vi "Tree Rows from Delimited String Array_csm.vi"(8 "Use Child Only? (F)":bool, 9 "Default Symbol":i32, 10 "Delimiter":string="\\", 11 "Items (Delimited)":string[][](array[string])) -> (2 "Parent Tag Added[]":string[](array[string]), 3 "Item to Add[]":T1(array[cluster]))   [LabVIEW 2017, in "csm-ui-support.lvlib"]
uses:
  csm-ui-support.lvlib
panel:
  out "Index":i32
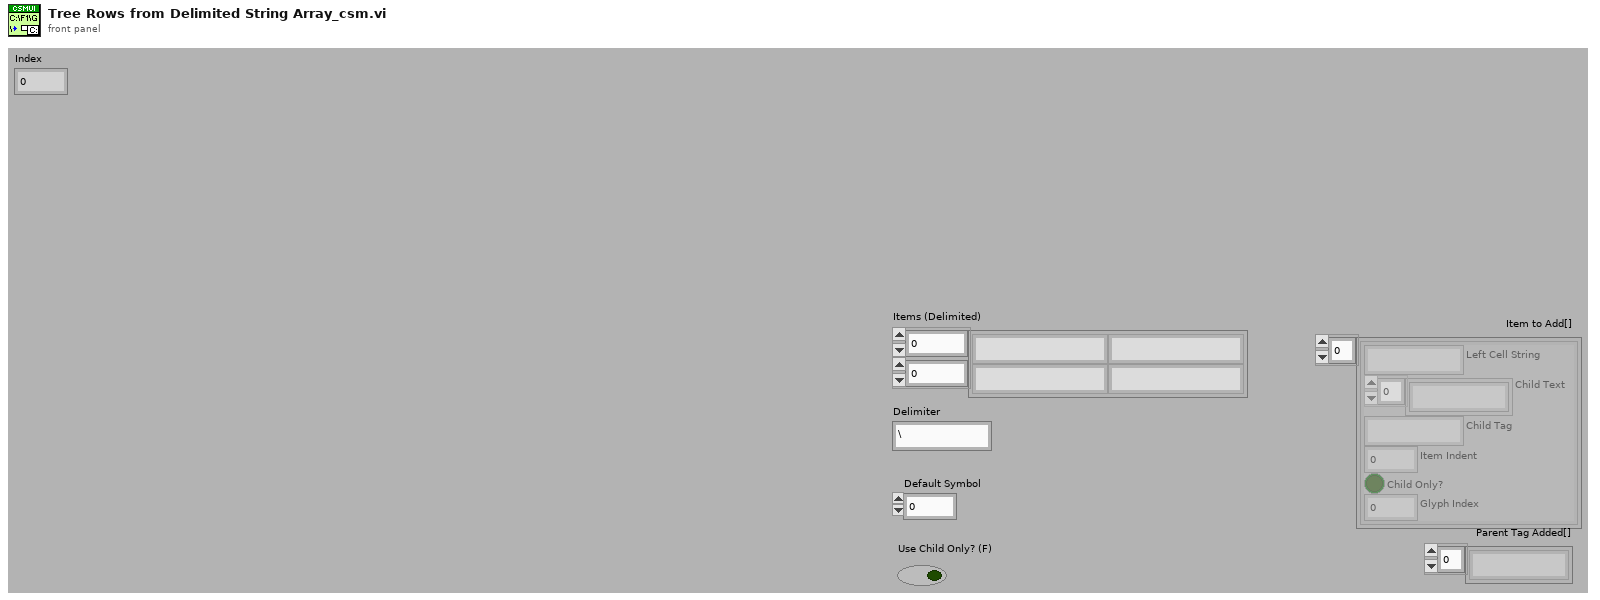
[diagram p1: front panel]
types:
  T1 = cluster{"Left Cell String":string, "Child Text":string[], "Child Tag":string, "Item Indent":i32, "Child Only?":bool, "Glyph Index":i32}[]
  T2 = cluster{"Left Cell String":string, "Child Text":string[], "Child Tag":string, "Item Indent":i32, "Child Only?":bool, "Glyph Index":i32}
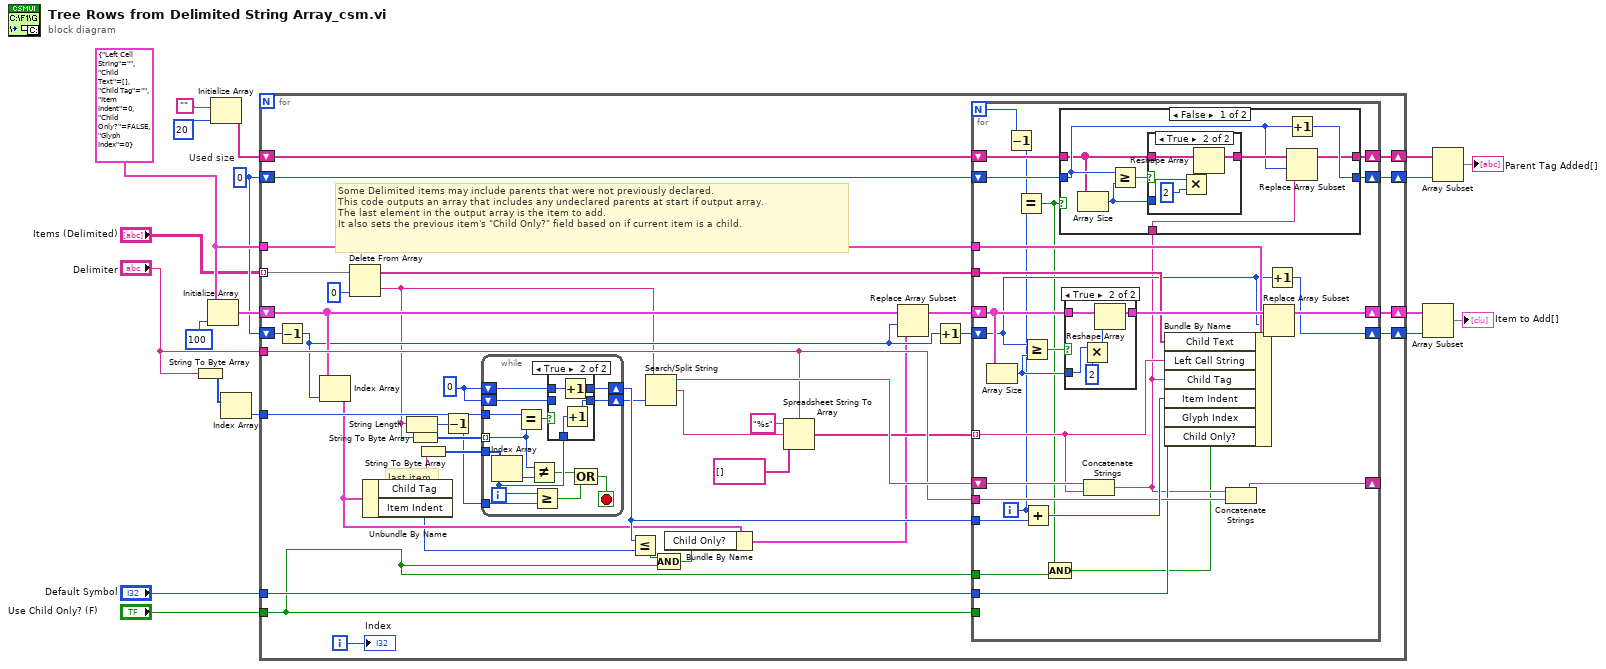
[diagram p0: block diagram]
diagram:
  w2 = 0  # Used size
  w8 = T2 {"Left Cell String"="", "Child Text"=[], "Child Tag"="", "Item Indent"=0, "Child Only?"=FALSE, "Glyph Index"=0} ("Item")
  n1 = String To Byte Array(string="Delimiter") -> (unsigned byte array=w18:u8[])
  n2 = Initialize Array(w8, 100 ("dimension size")) -> (w15:T1)
  n3 = Initialize Array("", 20 ("dimension size")) -> (w14:string[])
  n4 = Index Array(array=w18) -> (element=w19:u8)  [unwired: 1 in]
  n5 = for {
    shift-right: [w56] -> w17
    shift-left: w2 -> [w45]
    shift-right: [w57] -> w16
    shift-left: w15 -> [w46]
    tunnel: "Items (Delimited)" -> [w58] mode=indexing
    tunnel: "Delimiter" -> [w50]
    tunnel: w8 -> [w54]
    tunnel: w19 -> [w52]
    tunnel: "Default Symbol" -> [w47]
    tunnel: "Use Child Only? (F)" -> [w41]
    shift-right: [w38] -> w11
    shift-left: w14 -> [w40]
    shift-right: [w37] -> w10
    shift-left: w2 -> [w39]
    i -> [w53]
    w31 = 0
    # "last item"
    # "Some Delimited items may include parents that were not previously declared.\nThis code outputs an array that includes any undeclared parents at start if output array.\nThe last element in the output array is the item to add.\nIt also sets the previous item's \"Child Only?\" field based on if current item is a child."
    n6 = Decrement(x=w45) -> (x-1=w44:i32)
    n7 = Index Array(array=w46, index=w44) -> (element=w29:T2)
    n8 = Delete From Array(array=w58, index=0) -> (deleted portion=w24:string, array with subset deleted=w55:string[])  [unwired: 1 in]
    n9 = Unbundle By Name(w29) -> ("Child Tag"=w35:string, "Item Indent"=w26:i32)
    n10 = String Length(string=w24) -> (length=w23:i32)
    n11 = String To Byte Array(string=w24) -> (unsigned byte array=w34:u8[])
    n12 = String To Byte Array(string=w35) -> (unsigned byte array=w33:u8[])
    n13 = Decrement(x=w23) -> (x-1=w22:i32)
    n14 = while {
      shift-right: [w66] -> w48
      shift-left: w31 -> [w67]
      tunnel: w34 -> [w70] mode=indexing
      tunnel: w33 -> [w72]
      tunnel: w52 -> [w69]
      shift-right: [w65] -> w30
      shift-left: w31 -> [w64]
      tunnel: w22 -> [w62]
      i -> [w61]
      stop <- w63 stop-if-true
      n15 = Index Array(array=w72, index=w61) -> (element=w71:u8)
      n16 = Equal?(x=w69, y=w70) -> (x = y?=w68:bool)
      n17 = Not Equal?(x=w70, y=w71) -> (x != y?=w59:bool)
      n18 = Greater Or Equal?(x=w61, y=w62) -> (x >= y?=w60:bool)
      n19 = case shown="True" w68 {
        tunnel: w67 -> [w74 w78]
        tunnel: w64 -> [w73 _]
        tunnel: [w74 w77] -> w66
        tunnel: w61 -> [_ w76]
        tunnel: [w73 w75] -> w65
        frame False {
        }
        frame True {
          n20 = Increment(x=w78) -> (x+1=w77:i32)
          n21 = Increment(x=w76) -> (x+1=w75:i32)
        }
      }
      n22 = Compound Arithmetic op=OR(w59, w60) -> (w63:bool)
    }
    n23 = Less Or Equal?(x=w48, y=w26) -> (x <= y?=w25:bool)
    n24 = Search/Split String(string=w24, offset (0)=w30) -> (substring before match=w51:string, match + rest of string=w32:string)  [unwired: 1 in, 1 out]
    n25 = Compound Arithmetic op=AND(w25, w41) -> (w27:bool)
    n26 = Bundle By Name(cluster=w29, "Child Only?"=w27) -> (w28:T2)
    n27 = Spreadsheet String To Array(delimiter (Tab)=w50, format string="%s", spreadsheet string=w32, array type (2D Dbl)=string[] [] ("Array of Strings")) -> (array=w49:string[])
    n28 = Replace Array Subset(array=w46, new element=w28, index=w44) -> (w43:T1)
    n29 = Increment(x=w44) -> (x+1=w42:i32)
    n30 = for {
      N -> [w83]
      shift-right: [w103] -> w57
      shift-left: w43 -> [w106]
      shift-right: [w91] -> w56
      shift-left: w42 -> [w92]
      tunnel: w55 -> [w99]
      tunnel: w54 -> [w101]
      shift-right: [w95] -> _
      shift-left: w51 -> [w98]
      tunnel: w50 -> [w96]
      tunnel: w48 -> [w94]
      tunnel: w49 -> [w93] mode=indexing
      tunnel: w47 -> [w90]
      tunnel: w41 -> [_]
      tunnel: w41 -> [w80]
      shift-right: [w87] -> w38
      shift-left: w40 -> [w86]
      shift-right: [w88] -> w37
      shift-left: w39 -> [w89]
      i -> [w84]
      n31 = Array Size(array=w106) -> (size(s)=w104:i32)
      n32 = Decrement(x=w83) -> (x-1=w82:i32)
      n33 = Equal?(x=w82, y=w84) -> (x = y?=w81:bool)
      n34 = Greater Or Equal?(x=w92, y=w104) -> (x >= y?=w105:bool)
      n35 = Add(x=w84, y=w94) -> (x+y=w97:i32)
      n36 = Compound Arithmetic op=AND(w81, w80) -> (w79:bool)
      n37 = case shown="True" w105 {
        tunnel: w106 -> [w123 w126]
        tunnel: [w123 w128] -> w102
        tunnel: w104 -> [_ w124]
        frame False {
        }
        frame True {
          n38 = Multiply(x=w124, y=2) -> (x*y=w127:i32)
          n39 = Reshape Array(w126, w127) -> (w128:T1)
        }
      }
      n40 = Concatenate Strings(w98, w93) -> (w85:string)
      n41 = case shown="False" w81 {
        tunnel: w89 -> [w112 w121]
        tunnel: [w111 w121] -> w88
        tunnel: [w110 w122] -> w87
        tunnel: w86 -> [w108 w122]
        tunnel: w85 -> [w107 _]
        frame False {
          n42 = Array Size(array=w108) -> (size(s)=w114:i32)
          n43 = Greater Or Equal?(x=w112, y=w114) -> (x >= y?=w109:bool)
          n44 = case shown="True" w109 {
            tunnel: w108 -> [w115 w118]
            tunnel: [w115 w120] -> w113
            tunnel: w114 -> [_ w116]
            frame False {
            }
            frame True {
              n45 = Multiply(x=w116, y=2) -> (x*y=w119:i32)
              n46 = Reshape Array(w118, w119) -> (w120:string[])
            }
          }
          n47 = Increment(x=w112) -> (x+1=w111:i32)
          n48 = Replace Array Subset(array=w113, new element=w107, index=w112) -> (w110:string[])
        }
        frame True {
        }
      }
      n49 = Bundle By Name(cluster=w101, "Child Text"=w99, "Left Cell String"=w93, "Child Tag"=w85, "Item Indent"=w97, "Glyph Index"=w90, "Child Only?"=w79) -> (w100:T2)
      n50 = Concatenate Strings(w85, w96) -> (w95:string)
      n51 = Replace Array Subset(array=w102, new element=w100, index=w92) -> (w103:T1)
      n52 = Increment(x=w92) -> (x+1=w91:i32)
    }
    "Index" <- w53
  }
  n53 = Array Subset(array=w16, length=w17) -> (→"Item to Add[]":T1)  [unwired: 1 in]
  n54 = Array Subset(array=w11, length=w10) -> (→"Parent Tag Added[]":string[])  [unwired: 1 in]
